vi "Write to Indicator.vi"(11 "indicator data in":T1) -> (0 "error out":errorcluster, 3 "indicator data out":T1)   [LabVIEW 2018, in "GLog.lvlib" / "UI Updater.lvlib"]
uses:
  UI Updater.lvlib
  Indicator Data.ctl
panel:
  # "Connector Pane"
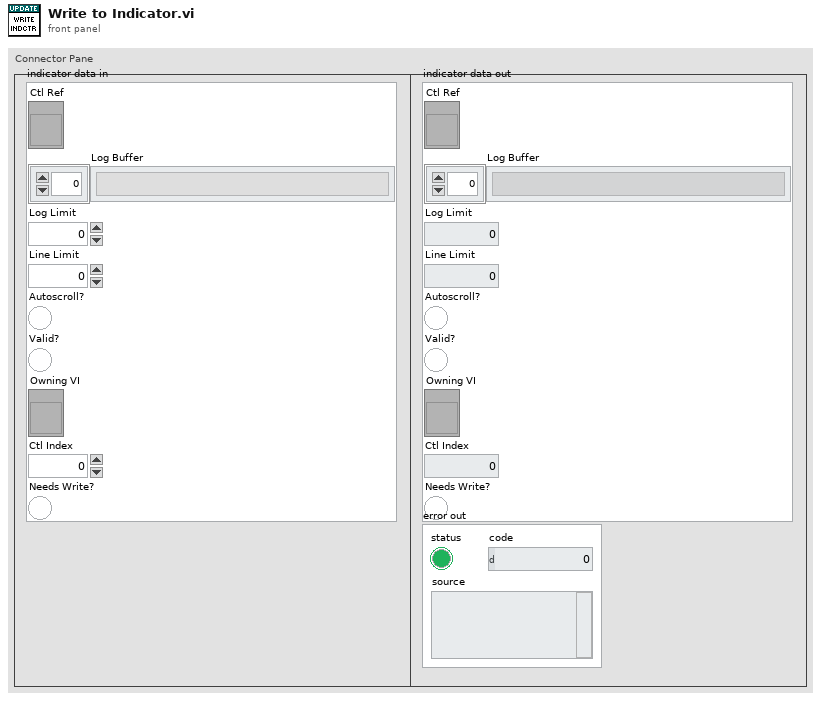
[diagram p1: front panel]
types:
  T1 = typedef "GLog.lvlib/UI Updater.lvlib/Indicator Data.ctl" = cluster{"Ctl Ref":refnum<vi>, "Log Buffer":string[], "Log Limit":i32, "Line Limit":i32, "Autoscroll?":bool, "Valid?":bool, "Owning VI":refnum<vi>, "Ctl Index":i32, "Needs Write?":bool}
  T2 = enum32{"Bad", "Idle", "Run top level", "Running"}
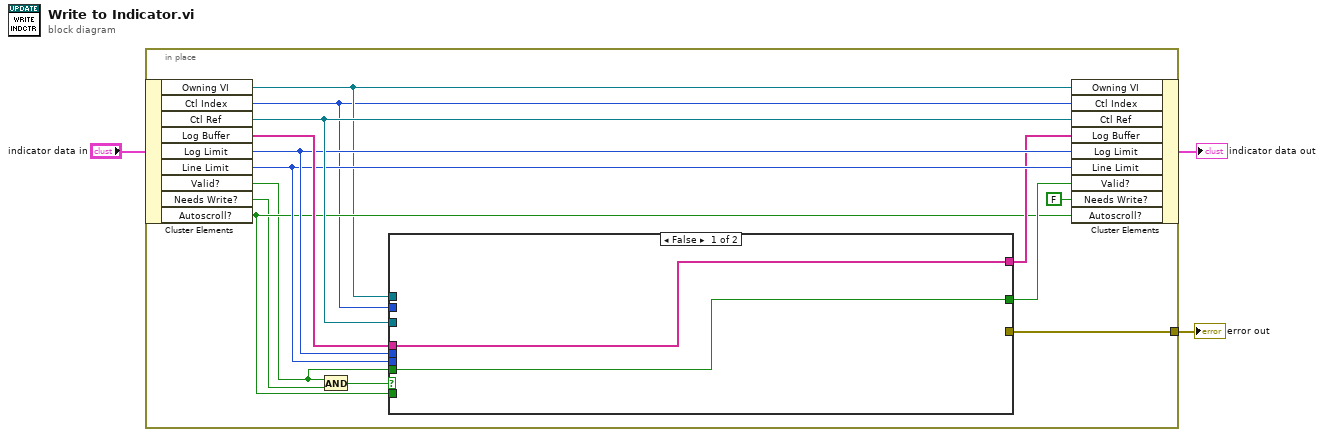
[diagram p0: block diagram]
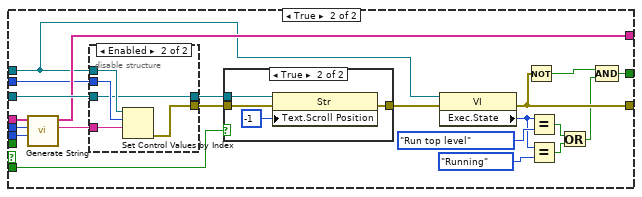
[diagram p2: hidden frame]
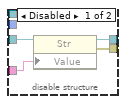
[diagram p3: hidden frame]
diagram:
  n1 = in-place {
    in-place-border: [w17] -> w1
    n2 = in-place-cluster #1("indicator data in") -> ("Owning VI"=w9:refnum<vi>, "Ctl Index"=w8:i32, "Ctl Ref"=w15:refnum<vi>, "Log Buffer"=w16:string[], "Log Limit"=w14:i32, "Line Limit"=w13:i32, "Valid?"=w4:bool, "Needs Write?"=w6:bool, "Autoscroll?"=w10:bool)
    n3 = And(x=w4, y=w6) -> (x .and. y?=w7:bool)
    n4 = case shown="False" w7 {
      tunnel: [_ w31] -> w17
      tunnel: w16 -> [w19 w40]
      tunnel: w15 -> [_ w39]
      tunnel: w14 -> [_ w38]
      tunnel: w13 -> [_ w37]
      tunnel: [w19 w35] -> w12
      tunnel: [w18 w24] -> w11
      tunnel: w10 -> [_ w32]
      tunnel: w9 -> [_ w20]
      tunnel: w8 -> [_ w22]
      tunnel: w4 -> [w18 _]
      frame False {
      }
      frame True {
        n5 = call "Generate String.vi"("line limit"=w37, "log limit"=w38, "log buffer"=w40) -> ("indicator string"=w36:string, "trimmed log buffer"=w35:string[])  [unwired: 7 in]
        n6 = disable-structure shown="Enabled" {
          disable-tunnel: w39 -> [w44 w45]
          disable-tunnel: w36 -> [w41 w46]
          disable-tunnel: [w43 w49] -> w34
          disable-tunnel: [w42 w45] -> w33
          disable-tunnel: w20 -> [_ w48]
          disable-tunnel: w22 -> [_ w47]
          frame Disabled {
            n7 = property class="Str"(reference=w44, "Value"=w41) -> (reference out=w42:refnum<vi>, error out=w43:errorcluster)  [unwired: 1 in]
          }
          frame Enabled {
            n8 = Set Control Values by Index(0:w48, 1:w47, 2:w46) -> (11:w49:errorcluster)  [unwired: 1 in]
          }
        }
        n9 = case shown="True" w32 {
          tunnel: w34 -> [w50 w54]
          tunnel: [w50 w53] -> w21
          tunnel: w33 -> [_ w52]
          frame False {
          }
          frame True {
            n10 = property class="Str"(reference=w52, error in=w54, "Text.Scroll Position"=-1) -> (error out=w53:errorcluster)  [unwired: 1 out]
          }
        }
        n11 = property class="VI"(reference=w20, error in=w21) -> (error out=w31:errorcluster, "Exec.State"=w29:T2)  [unwired: 1 out]
        n12 = Not(x=w31) -> (.not. x?=w25:bool)
        n13 = Equal?(x=w29, y=T2."Run top level") -> (x = y?=w27:bool)
        n14 = Equal?(x=w29, y=T2."Running") -> (x = y?=w26:bool)
        n15 = Or(x=w27, y=w26) -> (x .or. y?=w23:bool)
        n16 = Compound Arithmetic op=AND(w25, w23) -> (w24:bool)
      }
    }
    n17 = in-place-cluster #1("Owning VI"=w9, "Ctl Index"=w8, "Ctl Ref"=w15, "Log Buffer"=w12, "Log Limit"=w14, "Line Limit"=w13, "Valid?"=w11, "Needs Write?"=FALSE, "Autoscroll?"=w10) -> (→"indicator data out":T1)
  }
  "error out" <- w1
